vi "UE_Command_Permitted.vi"(8 "no_fault":bool, 9 "interlocks_satisfied":bool, 10 "resource_owned":bool, 11 "mode_authorized":bool) -> (3 "permitted":bool)   [LabVIEW 2026]
doc: "INTENT: Combine mode, resource ownership, interlock and fault checks for normal command authorization. INPUTS: mode_authorized (bool), resource_owned (bool), interlocks_satisfied (bool), no_fault (bool). OUTPUTS: permitted (bool). DESIGN CONSTRAINT: Decision helper only; bridge must also enforce ownership expiry, command identity, limits and target capability. REQUIREMENTS: SRS-F-021. No physical hardware side effects. Acceptance requires native LabVIEW compilation and behavioral testing."
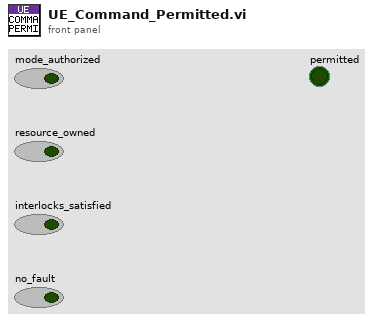
[diagram p1: front panel]
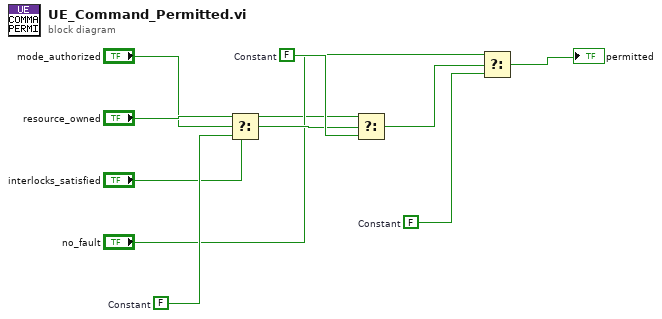
[diagram p0: block diagram]
diagram:
  w9 = FALSE  # Constant
  w7 = FALSE  # Constant
  w5 = FALSE  # Constant
  n1 = Select(t="resource_owned", s="mode_authorized", f=w5) -> (s? t:f=w6:bool)
  n2 = Select(t="interlocks_satisfied", s=w6, f=w7) -> (s? t:f=w8:bool)
  n3 = Select(t="no_fault", s=w8, f=w9) -> (s? t:f=→"permitted":bool)
